vi "Generate Client.vi"(8 "error in":errorcluster, 9 "client name":string, 10 "service class":string, 11 "project path":path) -> (0 "error out":errorcluster)   [LabVIEW 2021, in "NI Measurement V2 Client Generator Runtime.lvlib"]
doc: "Generates client for the measurement plug-in referred by the service class."
uses:
  NI Measurement V2 Client Generator Runtime.lvlib
  Client Generator Error Strings Global.vi
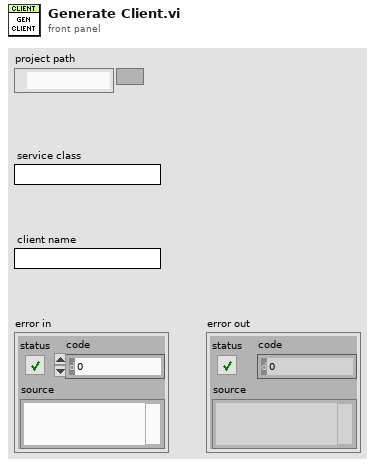
[diagram p1: front panel]
types:
  T1 = typedef "Measurement Service Client V2.lvlib/ni_measurementlink_measurement_v2_GetMetadataResponse.ctl" = cluster{"measurement_details":T2, "measurement_signature":T3, "user_interface_details":T10[]}
  T2 = typedef "Measurement Service Client V2.lvlib/ni_measurementlink_measurement_v2_MeasurementDetails.ctl" = cluster{"display_name":string, "version":string}
  T3 = typedef "Measurement Service Client V2.lvlib/ni_measurementlink_measurement_v2_MeasurementSignature.ctl" = cluster{"configuration_parameters_message_type":string, "configuration_parameters":T4[], "configuration_defaults":T7, "outputs_message_type":string, "outputs":T8[]}
  T4 = typedef "Measurement Service Client V2.lvlib/ni_measurementlink_measurement_v2_ConfigurationParameter.ctl" = cluster{"field_number":i32, "type":T5, "name":string, "repeated":bool, "annotations":T6[], "message_type":string}
  T5 = typedef "Measurement Service Client V2.lvlib/google_protobuf_Field_Kind.ctl" = enum32{"TYPE_UNKNOWN", "TYPE_DOUBLE", "TYPE_FLOAT", "TYPE_INT64", "TYPE_UINT64", "TYPE_INT32", "TYPE_FIXED64", "TYPE_FIXED32", "TYPE_BOOL", "TYPE_STRING", "TYPE_GROUP", "TYPE_MESSAGE", "TYPE_BYTES", "TYPE_UINT32", "TYPE_ENUM", "TYPE_SFIXED32", "TYPE_SFIXED64", "TYPE_SINT32", "TYPE_SINT64"}
  T6 = typedef "Measurement Service Client V2.lvlib/ni_measurementlink_measurement_v2_ConfigurationParameter_AnnotationsEntry.ctl" = cluster{"key":string, "value":string}
  T7 = typedef "Measurement Service Client V2.lvlib/google_protobuf_Any.ctl" = cluster{"type_url":string, "value":u8[]}
  T8 = typedef "Measurement Service Client V2.lvlib/ni_measurementlink_measurement_v2_Output.ctl" = cluster{"field_number":i32, "type":T5, "name":string, "repeated":bool, "annotations":T9[], "message_type":string}
  T9 = typedef "Measurement Service Client V2.lvlib/ni_measurementlink_measurement_v2_Output_AnnotationsEntry.ctl" = cluster{"key":string, "value":string}
  T10 = typedef "Measurement Service Client V2.lvlib/ni_measurementlink_measurement_v2_UserInterfaceDetails.ctl" = cluster{"file_url":string}
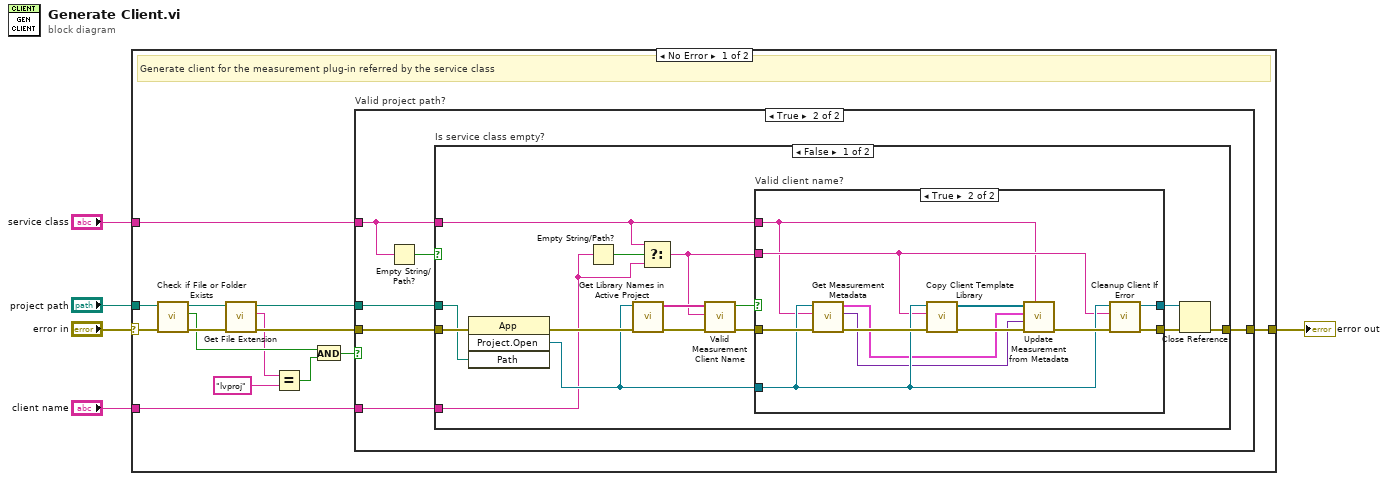
[diagram p0: block diagram]
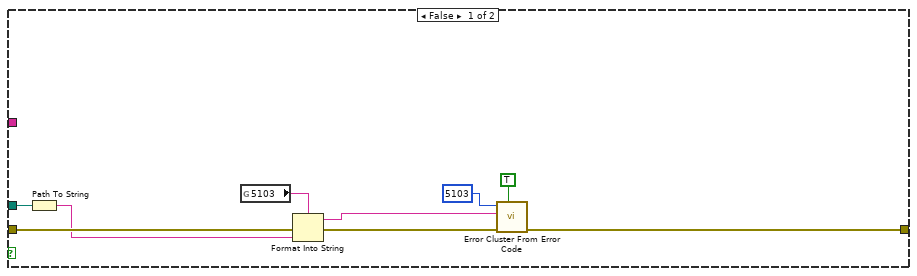
[diagram p2: hidden frame]
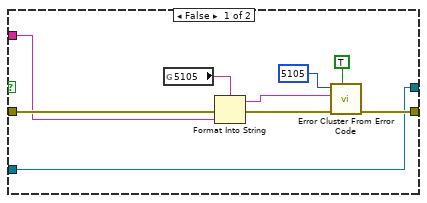
[diagram p3: hidden frame]
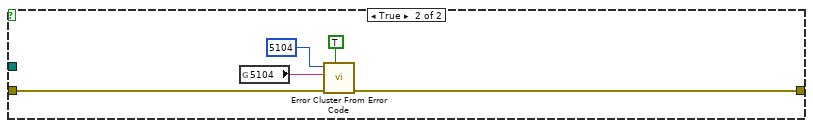
[diagram p4: hidden frame]
diagram:
  n1 = case shown="No Error" "error in" {
    selector: "error in" -> [w18 w76]
    tunnel: "service class" -> [w19 _]
    tunnel: [w8 w76] -> w1
    tunnel: "project path" -> [w15 _]
    tunnel: "client name" -> [w9 _]
    frame No Error {
      # "Generate client for the measurement plug-in referred by the service class"
      n2 = call <vilib>:"Check if File or Folder Exists.vi"("error in (no error)"=w18, "path"=w15) -> ("error out"=w17:errorcluster, "file or folder exists?"=w14:bool, "dup path"=w13:path)  [unwired: 7 in]
      n3 = call <vilib>:"Get File Extension.vi"("error in (no error)"=w17, "file"=w13) -> ("error out"=w16:errorcluster, "lowercase file extension"=w10:string, "dup file"=w12:path)  [unwired: 5 in, 2 out]
      n4 = Equal?(x=w10, y="lvproj") -> (x = y?=w7:bool)
      n5 = And(x=w14, y=w7) -> (x .and. y?=w6:bool)
      n6 = case "Valid project path?" shown="True" w6 {
        tunnel: w19 -> [_ w30]
        tunnel: [w27 w32] -> w8
        tunnel: w16 -> [w28 w34]
        tunnel: w12 -> [w23 w33]
        tunnel: w9 -> [_ w31]
        frame False {
          n7 = Path To String(path=w23) -> (string=w24:string)
          n8 = global read "Client Generator Error Strings Global.vi" "5103"() -> (w25:string)
          n9 = Format Into String(format string=w25, error in=w28, w24) -> (resulting string=w20:string, error out=w26:errorcluster)  [unwired: 1 in]
          n10 = call <vilib>:"Error Cluster From Error Code.vi"("show call chain? (False)"=TRUE, "error in (no error)"=w26, "error message (\"\")"=w20, "error code (0)"=5103) -> ("error out"=w27:errorcluster)  [unwired: 5 in]
        }
        frame True {
          n11 = Empty String/Path?(string/path=w30) -> (empty?=w29:bool)
          n12 = case "Is service class empty?" shown="False" w29 {
            tunnel: w34 -> [w49 w75]
            tunnel: w33 -> [w48 _]
            tunnel: [w41 w74] -> w32
            tunnel: w31 -> [w35 _]
            tunnel: w30 -> [w37 _]
            frame False {
              n13 = invoke class="App" method="Project.Open"(error in=w49, "Path"=w48) -> (error out=w39:errorcluster, "Project:Open"=w38:refnum<vi>)  [unwired: 2 in, 2 out]
              n14 = Empty String/Path?(string/path=w35) -> (empty?=w44:bool)
              n15 = call "Get Library Names in Active Project.vi"("error in (no error)"=w39, "project ref"=w38) -> ("error out"=w47:errorcluster, "library names"=w45:string[])  [unwired: 8 in]
              n16 = Select(t=w37, s=w44, f=w35) -> (s? t:f=w36:string)
              n17 = call "Valid Measurement Client Name.vi"("error in"=w47, "requested client name"=w36, "library names"=w45) -> ("error out"=w46:errorcluster, "valid name?"=w43:bool)  [unwired: 7 in]
              n18 = case "Valid client name?" shown="True" w43 {
                tunnel: [w53 w66] -> w40
                tunnel: [w57 w67] -> w42
                tunnel: w46 -> [w58 w65]
                tunnel: w37 -> [_ w61]
                tunnel: w38 -> [w53 w63]
                tunnel: w36 -> [w50 w62]
                frame False {
                  n19 = global read "Client Generator Error Strings Global.vi" "5105"() -> (w54:string)
                  n20 = Format Into String(format string=w54, error in=w58, w50) -> (resulting string=w55:string, error out=w56:errorcluster)  [unwired: 1 in]
                  n21 = call <vilib>:"Error Cluster From Error Code.vi"("show call chain? (False)"=TRUE, "error in (no error)"=w56, "error message (\"\")"=w55, "error code (0)"=5105) -> ("error out"=w57:errorcluster)  [unwired: 5 in]
                }
                frame True {
                  n22 = call "Get Measurement Metadata.vi"("error in"=w65, "service_class"=w61, "project refnum"=w63) -> ("error out"=w64:errorcluster, "default value"=w59:variant, "metadata"=w60:T1)  [unwired: 6 in]
                  n23 = call "Copy Client Template Library.vi"("error in"=w64, "new library name"=w62, "project ref"=w63) -> ("error out"=w70:errorcluster, "file refnums"=w68:refnum<vi>[])  [unwired: 7 in]
                  n24 = call "Update Measurement from Metadata.vi"("client service_class"=w61, "error in"=w70, "default value"=w59, "metadata"=w60, "file refnums"=w68) -> ("error out"=w69:errorcluster)  [unwired: 6 in]
                  n25 = call "Cleanup Client If Error.vi"("error in"=w69, "client name"=w62, "project ref in"=w63) -> ("error out"=w67:errorcluster, "project ref out"=w66:refnum<vi>)  [unwired: 7 in]
                }
              }
              n26 = Close Reference(reference=w40, error in (no error)=w42) -> (error out=w41:errorcluster)
            }
            frame True {
              n27 = global read "Client Generator Error Strings Global.vi" "5104"() -> (w72:string)
              n28 = call <vilib>:"Error Cluster From Error Code.vi"("show call chain? (False)"=TRUE, "error in (no error)"=w75, "error message (\"\")"=w72, "error code (0)"=5104) -> ("error out"=w74:errorcluster)  [unwired: 5 in]
            }
          }
        }
      }
    }
    frame Error {
      # "Pass"
    }
  }
  "error out" <- w1
